vi "Build Wiring Spec.vi"(8 "error in (no error)":errorcluster, 10 "References":T1) -> (0 "error out":errorcluster, 4 "Wiring Spec":T2)   [LabVIEW 2023, in "Message Maker.lvclass"]
doc: "Figures out the wiring spec for the new message. This wiring spec is used to build the new message\n\nAuthor: Derek Trepanier\nCopyright: MGI 2015"
uses:
  Message Maker.lvclass
  Wiring Spec.ctl
  Connector Pane Position.ctl
  Scripting Refs.ctl
  Message Maker.lvclass/Message Maker.ctl
  <vilib>/Utility/Data Type/NI_Data Type.lvlib
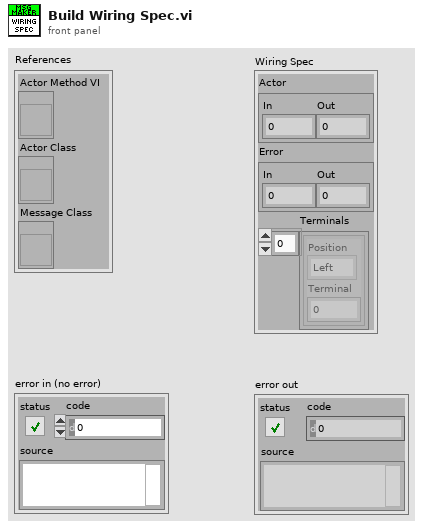
[diagram p1: front panel]
types:
  T1 = typedef "Message Maker.lvclass/Scripting Refs.ctl" = cluster{"Actor Method VI":refnum<vi>, "Actor Class":refnum<vi>, "Message Class":refnum<vi>}
  T2 = typedef "Message Maker.lvclass/Wiring Spec.ctl" = cluster{"Actor":cluster{"In":i32, "Out":i32}, "Error":cluster{"In":i32, "Out":i32}, "Terminals":cluster{"Position":T3, "Terminal":i32}[]}
  T3 = typedef "Message Maker.lvclass/Connector Pane Position.ctl" = enum16{"Left", "Top", "Bottom", "Right"}
  T4 = cluster{"Actor":cluster{"In":i32, "Out":i32}, "Error":cluster{"In":i32, "Out":i32}, "Left":cluster{"Position":i16, "Terminal":i32}[], "Bottom":cluster{"Position":i16, "Terminal":i32}[], "Right":cluster{"Position":i16, "Terminal":i32}[], "Top":cluster{"Position":i16, "Terminal":i32}[]}
  T5 = typedef "LVRectTypeDef.ctl" = cluster{"Left":i16, "Top":i16, "Right":i16, "Bottom":i16}
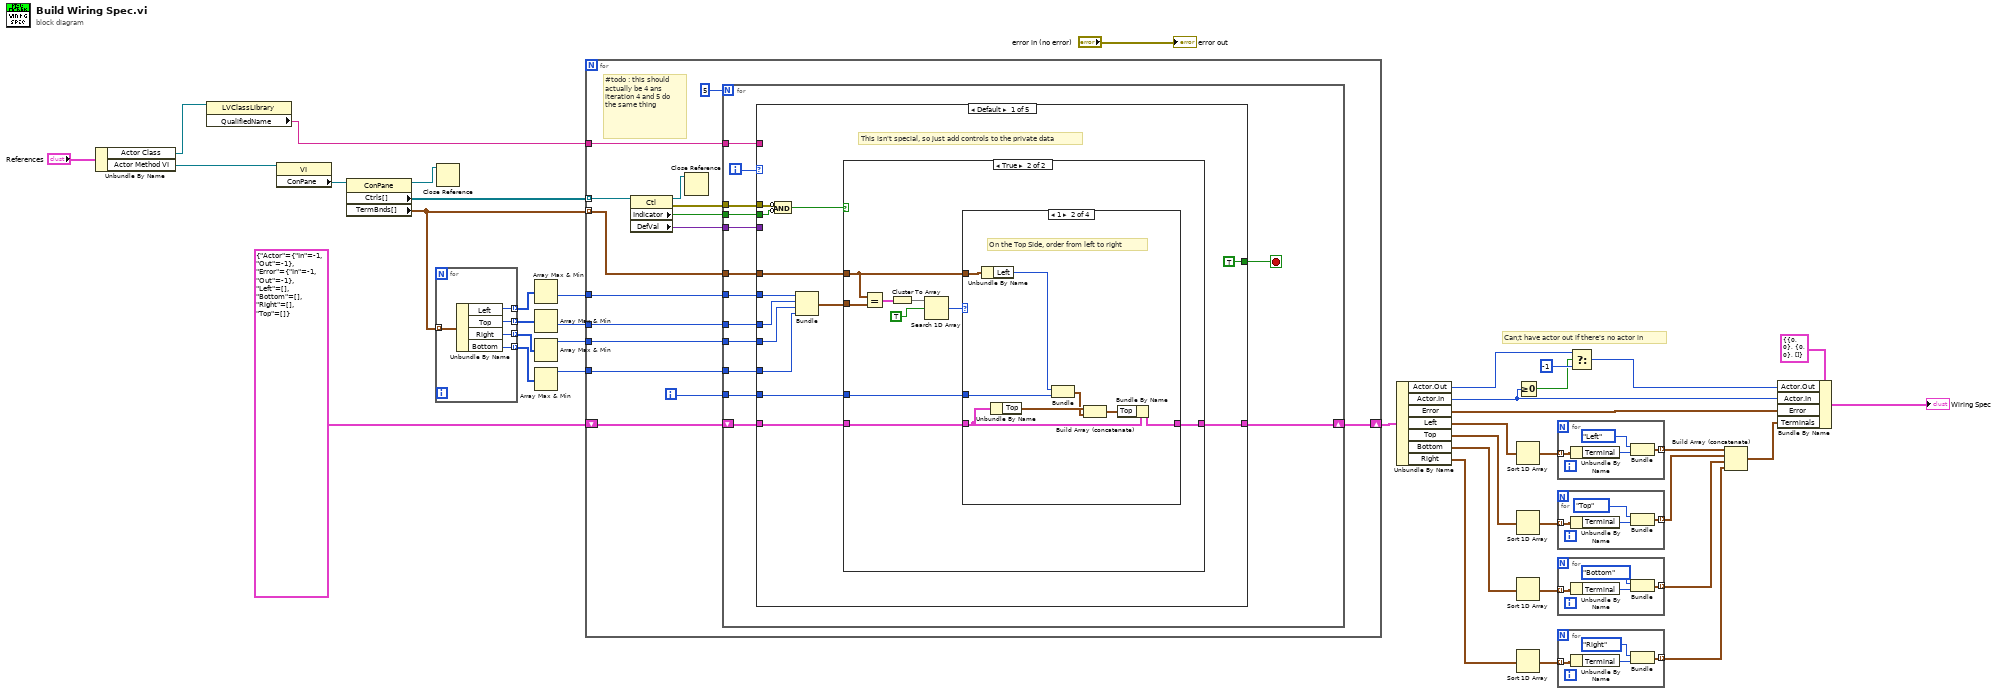
[diagram p0: block diagram]
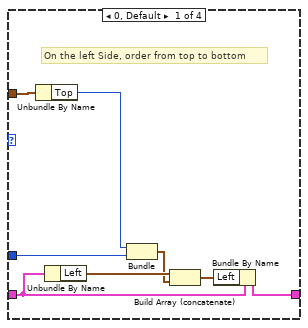
[diagram p3: hidden frame]
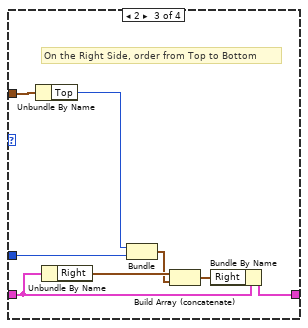
[diagram p4: hidden frame]
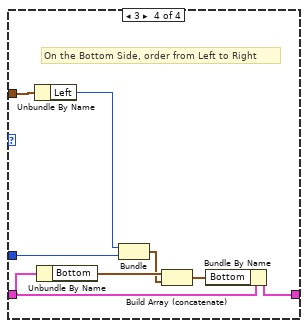
[diagram p5: hidden frame]
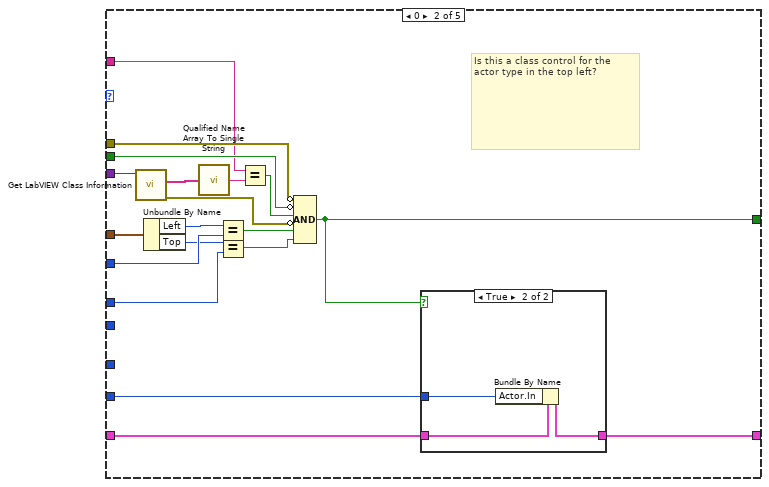
[diagram p6: hidden frame]
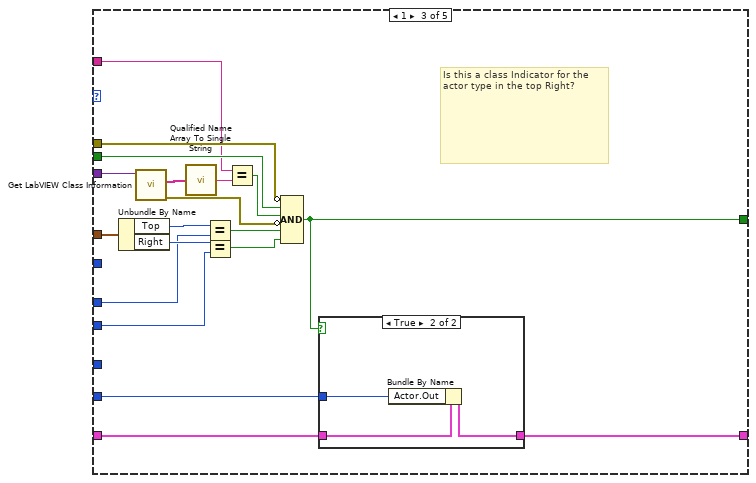
[diagram p8: hidden frame]
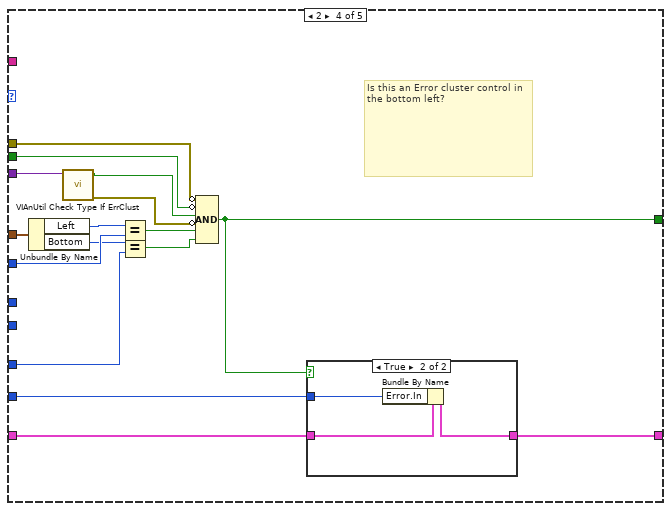
[diagram p10: hidden frame]
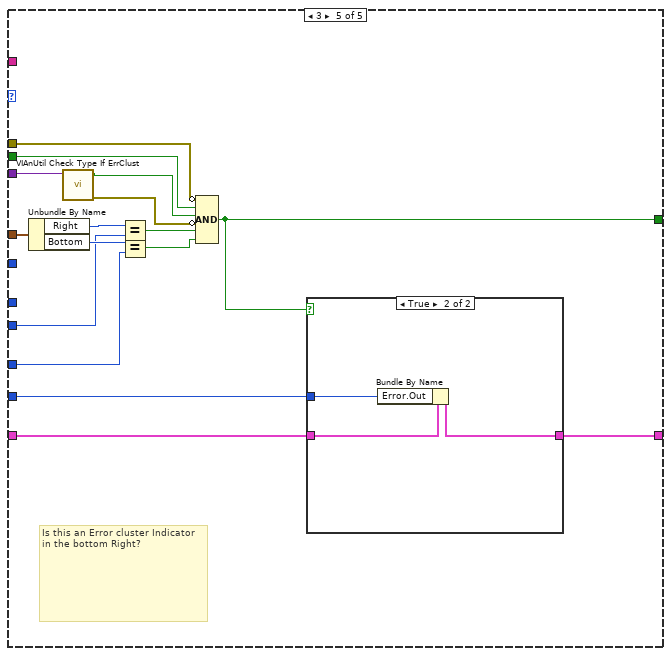
[diagram p12: hidden frame]
diagram:
  # "Can;t have actor out if there's no actor in"
  n1 = Unbundle By Name("References") -> ("Actor Class"=w4:refnum<vi>, "Actor Method VI"=w2:refnum<vi>)
  n2 = property class="LVClassLibrary"(reference=w4) -> ("QualifiedName"=w3:string)  [unwired: 1 in, 2 out]
  n3 = property class="VI"(reference=w2) -> ("ConPane"=w40:refnum<vi>)  [unwired: 1 in, 2 out]
  n4 = property class="ConPane"(reference=w40) -> (reference out=w29:refnum<vi>, "Ctrls[]"=w39:refnum<vi>[], "TermBnds[]"=w38:T5[])  [unwired: 1 in, 1 out]
  n5 = for {
    tunnel: w38 -> [w45] mode=indexing
    tunnel: [w44] -> w37 mode=indexing
    tunnel: [w43] -> w36 mode=indexing
    tunnel: [w42] -> w35 mode=indexing
    tunnel: [w41] -> w34 mode=indexing
    n6 = Unbundle By Name(w45) -> ("Left"=w44:i16, "Top"=w43:i16, "Right"=w42:i16, "Bottom"=w41:i16)
  }
  n7 = Close Reference(reference=w29) -> ()  [unwired: 1 in, 1 out]
  n8 = Array Max & Min(array=w37) -> (min value=w33:i16)  [unwired: 3 out]
  n9 = Array Max & Min(array=w36) -> (min value=w32:i16)  [unwired: 3 out]
  n10 = Array Max & Min(array=w35) -> (max value=w31:i16)  [unwired: 3 out]
  n11 = Array Max & Min(array=w34) -> (max value=w30:i16)  [unwired: 3 out]
  n12 = for {
    tunnel: w39 -> [w60] mode=indexing
    tunnel: w38 -> [w58] mode=indexing
    tunnel: w33 -> [w57]
    tunnel: w32 -> [w56]
    tunnel: w31 -> [w49]
    tunnel: w30 -> [w50]
    tunnel: w3 -> [w52]
    shift-right: [w46] -> w27
    shift-left: T4 {"Actor"={"In"=-1, "Out"=-1}, "Error"={"In"=-1, "Out"=-1}, "Left"=[], "Bottom"=[], "Right"=[], "Top"=[]} -> [w47]
    i -> [w51]
    # "#todo : this should actually be 4 ans iteration 4 and 5 do the same thing"
    # "Find Top Left, Bottom left controls AND\nTop Right and bottom right Indicators"
    n13 = property class="Ctl"(reference=w60) -> (reference out=w48:refnum<vi>, error out=w55:errorcluster, "Indicator"=w54:bool, "DefVal"=w53:variant)  [unwired: 1 in]
    n14 = Close Reference(reference=w48) -> ()  [unwired: 1 in, 1 out]
    n15 = for {
      N: 5 -> [_]
      tunnel: w58 -> [w73]
      shift-right: [w64] -> w46
      shift-left: w47 -> [w72]
      tunnel: w57 -> [w71]
      tunnel: w56 -> [w70]
      tunnel: w55 -> [w69]
      tunnel: w54 -> [w68]
      tunnel: w53 -> [w67]
      tunnel: w52 -> [w66]
      tunnel: w51 -> [w65]
      tunnel: w50 -> [w63]
      tunnel: w49 -> [w62]
      i -> [w74]
      stop <- w61 stop-if-true
      n16 = case shown="Default" w74 {
        tunnel: w73 -> [w80 w148 w171 w191 w211]
        tunnel: w72 -> [w87 w136 w158 w177 w197]
        tunnel: w71 -> [w79 w146 _ w189 _]
        tunnel: w70 -> [w78 w144 w156 _ _]
        tunnel: w69 -> [w85 w143 w168 w187 w208]
        tunnel: w68 -> [w84 w142 w167 w186 w207]
        tunnel: w67 -> [_ w132 w163 w182 w203]
        tunnel: w66 -> [_ w138 w160 _ _]
        tunnel: w65 -> [w82 w135 w157 w183 w204]
        tunnel: [w86 w133 w153 w176 w196] -> w64
        tunnel: w63 -> [w76 _ _ w179 w200]
        tunnel: w62 -> [w77 _ w155 _ w199]
        tunnel: [TRUE w134 w154 w178 w198] -> w61
        frame Default {
          # "This isn't special, so just add controls to the private data"
          n17 = Compound Arithmetic op=AND(invert w85, invert w84) -> (w83:bool)
          n18 = Bundle(w79, w78, w77, w76) -> (w75:cluster{i16, i16, i16, i16})  [unwired: 1 in]
          n19 = case shown="True" w83 {
            tunnel: w87 -> [w88 w91]
            tunnel: [w88 w89] -> w86
            tunnel: w82 -> [_ w90]
            tunnel: w80 -> [_ w92]
            tunnel: w75 -> [_ w97]
            frame False {
            }
            frame True {
              n20 = Equal?(x=w92, y=w97) -> (x = y?=w96:cluster{bool, bool, bool, bool})
              n21 = Cluster To Array(cluster=w96) -> (array=w95:bool[])
              n22 = Search 1D Array(1D array=w95, element=TRUE) -> (index of element=w93:i32)  [unwired: 1 in]
              n23 = case shown="1" w93 {
                tunnel: w92 -> [w105 w113 w121 w129]
                tunnel: w91 -> [w102 w110 w118 w126]
                tunnel: w90 -> [w103 w111 w119 w127]
                tunnel: [w99 w107 w115 w123] -> w89
                frame 0, Default {
                  # "On the left Side, order from top to bottom"
                  n24 = Unbundle By Name(w105) -> ("Top"=w104:i16)
                  n25 = Unbundle By Name(w102) -> ("Left"=w101:cluster{"Position":i16, "Terminal":i32}[])
                  n26 = Bundle("Top"=w104, w103) -> (w100:cluster{"Top":i16, i32})  [unwired: 1 in]
                  n27 = Build Array (concatenate)(w101, w100) -> (w98:cluster{"Top":i16, "Terminal":i32}[])
                  n28 = Bundle By Name(cluster=w102, "Left"=w98) -> (w99:T4)
                }
                frame 1 {
                  # "On the Top Side, order from left to right"
                  n29 = Unbundle By Name(w113) -> ("Left"=w112:i16)
                  n30 = Unbundle By Name(w110) -> ("Top"=w109:cluster{"Position":i16, "Terminal":i32}[])
                  n31 = Bundle("Left"=w112, w111) -> (w108:cluster{"Left":i16, i32})  [unwired: 1 in]
                  n32 = Build Array (concatenate)(w109, w108) -> (w106:cluster{"Left":i16, "Terminal":i32}[])
                  n33 = Bundle By Name(cluster=w110, "Top"=w106) -> (w107:T4)
                }
                frame 2 {
                  # "On the Right Side, order from Top to Bottom"
                  n34 = Unbundle By Name(w121) -> ("Top"=w120:i16)
                  n35 = Unbundle By Name(w118) -> ("Right"=w117:cluster{"Position":i16, "Terminal":i32}[])
                  n36 = Bundle("Top"=w120, w119) -> (w116:cluster{"Top":i16, i32})  [unwired: 1 in]
                  n37 = Build Array (concatenate)(w117, w116) -> (w114:cluster{"Top":i16, "Terminal":i32}[])
                  n38 = Bundle By Name(cluster=w118, "Right"=w114) -> (w115:T4)
                }
                frame 3 {
                  # "On the Bottom Side, order from Left to Right"
                  n39 = Unbundle By Name(w129) -> ("Left"=w128:i16)
                  n40 = Unbundle By Name(w126) -> ("Bottom"=w125:cluster{"Position":i16, "Terminal":i32}[])
                  n41 = Bundle("Left"=w128, w127) -> (w124:cluster{"Left":i16, i32})  [unwired: 1 in]
                  n42 = Build Array (concatenate)(w125, w124) -> (w122:cluster{"Left":i16, "Terminal":i32}[])
                  n43 = Bundle By Name(cluster=w126, "Bottom"=w122) -> (w123:T4)
                }
              }
            }
          }
        }
        frame 0 {
          # "Is this a class control for the actor type in the top left?"
          # "Top Left Actor Class Ctrl?"
          n44 = call <vilib>:"Get LabVIEW Class Information.vi"("variant"=w132) -> ("error out"=w130:errorcluster, "qualified LabVIEW class name"=w131:string[])  [unwired: 8 in, 1 out]
          n45 = Unbundle By Name(w148) -> ("Left"=w147:i16, "Top"=w145:i16)
          n46 = call <vilib>:"Qualified Name Array To Single String.vi"("Fully Qualified Array"=w131) -> ("Fully Qualified String"=w139:string)
          n47 = Equal?(x=w147, y=w146) -> (x = y?=w141:bool)
          n48 = Equal?(x=w145, y=w144) -> (x = y?=w140:bool)
          n49 = Equal?(x=w138, y=w139) -> (x = y?=w137:bool)
          n50 = Compound Arithmetic op=AND(invert w143, invert w142, w137, invert w130, w141, w140) -> (w134:bool)
          n51 = case shown="True" w134 {
            tunnel: w136 -> [w149 w150]
            tunnel: w135 -> [_ w151]
            tunnel: [w149 w152] -> w133
            frame False {
            }
            frame True {
              n52 = Bundle By Name(cluster=w150, "Actor.In"=w151) -> (w152:T4)
            }
          }
        }
        frame 1 {
          # "Is this a class Indicator for the actor type in the top Right?"
          # "Top Left Actor Class Ctrl?"
          n53 = Unbundle By Name(w171) -> ("Top"=w170:i16, "Right"=w169:i16)
          n54 = call <vilib>:"Get LabVIEW Class Information.vi"("variant"=w163) -> ("error out"=w162:errorcluster, "qualified LabVIEW class name"=w164:string[])  [unwired: 8 in, 1 out]
          n55 = call <vilib>:"Qualified Name Array To Single String.vi"("Fully Qualified Array"=w164) -> ("Fully Qualified String"=w161:string)
          n56 = Equal?(x=w170, y=w156) -> (x = y?=w166:bool)
          n57 = Equal?(x=w169, y=w155) -> (x = y?=w165:bool)
          n58 = Equal?(x=w160, y=w161) -> (x = y?=w159:bool)
          n59 = Compound Arithmetic op=AND(invert w168, w167, w159, invert w162, w166, w165) -> (w154:bool)
          n60 = case shown="True" w154 {
            tunnel: w158 -> [w172 w173]
            tunnel: w157 -> [_ w174]
            tunnel: [w172 w175] -> w153
            frame False {
            }
            frame True {
              n61 = Bundle By Name(cluster=w173, "Actor.Out"=w174) -> (w175:T4)
            }
          }
        }
        frame 2 {
          # "Is this an Error cluster control in the bottom left?"
          # "Top Left Actor Class Ctrl?"
          n62 = Unbundle By Name(w191) -> ("Left"=w190:i16, "Bottom"=w188:i16)
          n63 = call <vilib>:"VIAnUtil Check Type If ErrClust.vi"("Data In"=w182) -> ("error out"=w181:errorcluster, "IsErrClust?"=w180:bool)  [unwired: 9 in]
          n64 = Equal?(x=w190, y=w189) -> (x = y?=w185:bool)
          n65 = Equal?(x=w188, y=w179) -> (x = y?=w184:bool)
          n66 = Compound Arithmetic op=AND(invert w187, invert w186, w180, invert w181, w185, w184) -> (w178:bool)
          n67 = case shown="True" w178 {
            tunnel: w183 -> [_ w194]
            tunnel: [w192 w195] -> w176
            tunnel: w177 -> [w192 w193]
            frame False {
            }
            frame True {
              n68 = Bundle By Name(cluster=w193, "Error.In"=w194) -> (w195:T4)
            }
          }
        }
        frame 3 {
          # "Is this an Error cluster Indicator in the bottom Right?"
          # "Top Left Actor Class Ctrl?"
          n69 = Unbundle By Name(w211) -> ("Right"=w210:i16, "Bottom"=w209:i16)
          n70 = call <vilib>:"VIAnUtil Check Type If ErrClust.vi"("Data In"=w203) -> ("error out"=w202:errorcluster, "IsErrClust?"=w201:bool)  [unwired: 9 in]
          n71 = Equal?(x=w210, y=w199) -> (x = y?=w206:bool)
          n72 = Equal?(x=w209, y=w200) -> (x = y?=w205:bool)
          n73 = Compound Arithmetic op=AND(invert w208, w207, w201, invert w202, w206, w205) -> (w198:bool)
          n74 = case shown="True" w198 {
            tunnel: w204 -> [_ w214]
            tunnel: [w212 w215] -> w196
            tunnel: w197 -> [w212 w213]
            frame False {
            }
            frame True {
              n75 = Bundle By Name(cluster=w213, "Error.Out"=w214) -> (w215:T4)
            }
          }
        }
      }
    }
  }
  n76 = Unbundle By Name(w27) -> ("Actor.Out"=w23:i32, "Actor.In"=w20:i32, "Error"=w25:cluster{"In":i32, "Out":i32}, "Left"=w19:cluster{"Position":i16, "Terminal":i32}[], "Top"=w13:cluster{"Position":i16, "Terminal":i32}[], "Bottom"=w12:cluster{"Position":i16, "Terminal":i32}[], "Right"=w11:cluster{"Position":i16, "Terminal":i32}[])
  n77 = Sort 1D Array(array=w19) -> (sorted array=w18:cluster{"Position":i16, "Terminal":i32}[])
  n78 = Sort 1D Array(array=w13) -> (sorted array=w16:cluster{"Position":i16, "Terminal":i32}[])
  n79 = Sort 1D Array(array=w12) -> (sorted array=w15:cluster{"Position":i16, "Terminal":i32}[])
  n80 = Sort 1D Array(array=w11) -> (sorted array=w14:cluster{"Position":i16, "Terminal":i32}[])
  n81 = Greater Or Equal To 0?(x=w20) -> (x >= 0?=w21:bool)
  n82 = for {
    tunnel: w18 -> [w219] mode=indexing
    tunnel: [w216] -> w10 mode=indexing
    n83 = Unbundle By Name(w219) -> ("Terminal"=w217:i32)
    n84 = Bundle("Position"=Connector_Pane_Position."Left", "Terminal"=w217) -> (w216:cluster{"Position":T3, "Terminal":i32})  [unwired: 1 in]
  }
  n85 = for {
    tunnel: w16 -> [w223] mode=indexing
    tunnel: [w220] -> w9 mode=indexing
    n86 = Unbundle By Name(w223) -> ("Terminal"=w221:i32)
    n87 = Bundle("Position"=Connector_Pane_Position."Top", "Terminal"=w221) -> (w220:cluster{"Position":T3, "Terminal":i32})  [unwired: 1 in]
  }
  n88 = for {
    tunnel: w15 -> [w227] mode=indexing
    tunnel: [w224] -> w8 mode=indexing
    n89 = Unbundle By Name(w227) -> ("Terminal"=w225:i32)
    n90 = Bundle("Position"=Connector_Pane_Position."Bottom", "Terminal"=w225) -> (w224:cluster{"Position":T3, "Terminal":i32})  [unwired: 1 in]
  }
  n91 = for {
    tunnel: w14 -> [w231] mode=indexing
    tunnel: [w228] -> w7 mode=indexing
    n92 = Unbundle By Name(w231) -> ("Terminal"=w229:i32)
    n93 = Bundle("Position"=Connector_Pane_Position."Right", "Terminal"=w229) -> (w228:cluster{"Position":T3, "Terminal":i32})  [unwired: 1 in]
  }
  n94 = Select(t=w23, s=w21, f=-1) -> (s? t:f=w24:i32)
  n95 = Build Array (concatenate)(w10, w9, w8, w7) -> (w6:cluster{"Position":T3, "Terminal":i32}[])
  n96 = Bundle By Name(cluster=T2 {"Actor"={"In"=0, "Out"=0}, "Error"={"In"=0, "Out"=0}, "Terminals"=[]} ("Wiring Spec"), "Actor.Out"=w24, "Actor.In"=w20, "Error"=w25, "Terminals"=w6) -> (→"Wiring Spec":T2)
  "error out" <- "error in (no error)"
